vi "Populate Menu Activation.vi"(8 "error in (no error)":errorcluster, 9 "Coords":T1, 10 "MenuRef":refnum<k9>, 11 "Selector in":refnum<class "Selector.lvclass">) -> (0 "error out":errorcluster, 3 "Selector out":refnum<class "Selector.lvclass">)   [LabVIEW 2019, in "Selector.lvclass"]
uses:
  Selector.lvclass
  <vilib>/Utility/miscctls.llb/LVPoint32TypeDef.ctl
  Selector.lvclass/Selector.ctl
  f1f0a02b-b8b6-4cc5-b4ed-f95812147d19.vi
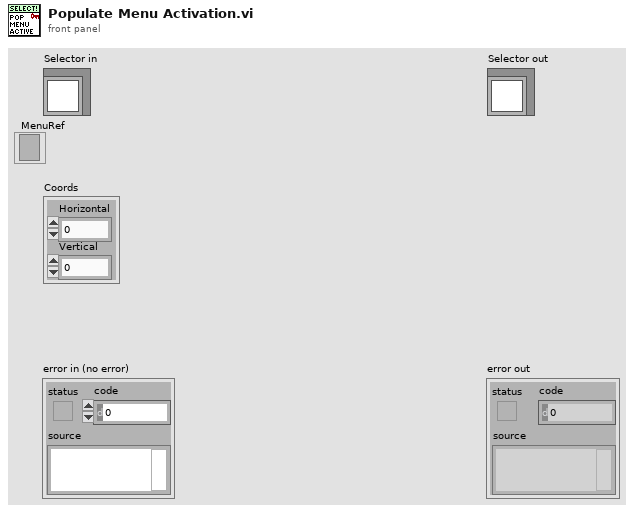
[diagram p1: front panel]
types:
  T1 = typedef "LVPoint32TypeDef.ctl" = cluster{"Horizontal":i32, "Vertical":i32}
  T2 = typedef "Selector.lvclass/Item.ctl" = cluster{"Name":string, "Group":string, "Enabled":bool}
  T3 = typedef "LVRowAndColumnTypeDef.ctl" = cluster{"Row":i32, "Column":i32}
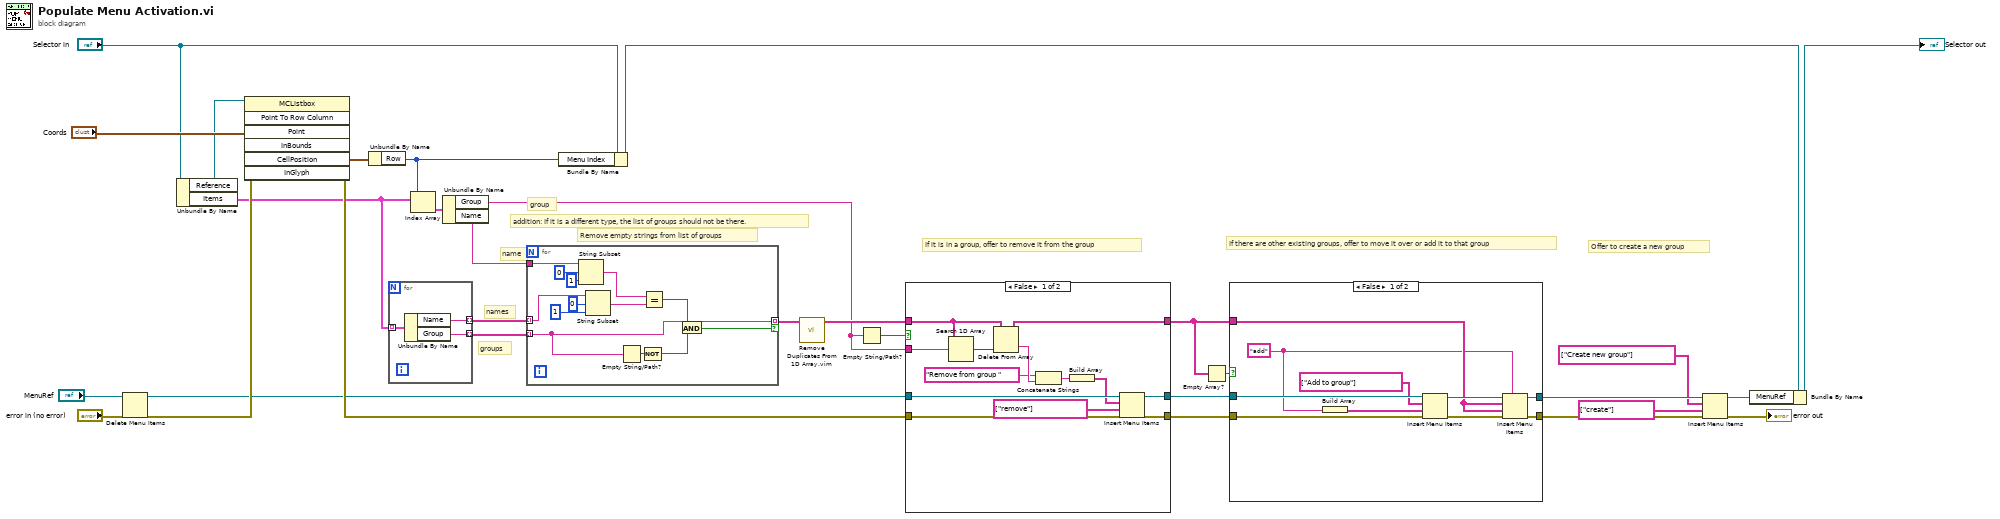
[diagram p0: block diagram]
diagram:
  # "group"
  # "name"
  # "groups"
  # "names"
  # "Remove empty strings from list of groups"
  # "addition: If it is a different type, the list of groups should not be there."
  # "Offer to create a new group"
  # "If there are other existing groups, offer to move it over or add it to that group"
  # "If it is in a group, offer to remove it from the group"
  n1 = Delete Menu Items(6:"error in (no error)", 9:"MenuRef") -> (0:w27:errorcluster, 3:w24:refnum<k9>)  [unwired: 2 in]
  n2 = Unbundle By Name("Selector in") -> ("Reference"=w14:refnum<vi>, "Items"=w3:T2[])
  n3 = invoke class="MCListbox" method="Point To Row Column"(reference=w14, error in=w27, "Point"="Coords") -> (error out=w25:errorcluster, "CellPosition"=w28:T3)  [unwired: 4 in, 5 out]
  n4 = Unbundle By Name(w28) -> ("Row"=w7:i32)
  n5 = for {
    tunnel: w3 -> [w34] mode=indexing
    tunnel: [w33] -> w2 mode=indexing
    tunnel: [w32] -> w1 mode=indexing
    n6 = Unbundle By Name(w34) -> ("Name"=w33:string, "Group"=w32:string)
  }
  n7 = Index Array(array=w3, index=w7) -> (element=w6:T2)
  n8 = Unbundle By Name(w6) -> ("Group"=w4:string, "Name"=w5:string)
  n9 = for {
    tunnel: w5 -> [w47]
    tunnel: [w36] -> w8 mode=indexing if=w35
    tunnel: w2 -> [w38] mode=indexing
    tunnel: w1 -> [w36] mode=indexing
    n10 = String Subset(string=w47, offset (0)=0, length (rest)=1 ("length (rest)")) -> (substring=w41:string)
    n11 = String Subset(string=w38, offset (0)=0, length (rest)=1 ("length (rest)")) -> (substring=w42:string)
    n12 = Empty String/Path?(string/path=w36) -> (empty?=w40:bool)
    n13 = Not(x=w40) -> (.not. x?=w39:bool)
    n14 = Equal?(x=w41, y=w42) -> (x = y?=w37:bool)
    n15 = And(x=w37, y=w39) -> (x .and. y?=w35:bool)
  }
  n16 = Bundle By Name(cluster="Selector in", "Menu Index"=w7) -> (w11:refnum<class "Selector.lvclass">)
  n17 = call "Remove Duplicates From 1D Array.vim"("array"=w8) -> ("array with duplicates removed"=w9:string[])  [unwired: 10 in]
  n18 = Empty String/Path?(string/path=w4) -> (empty?=w26:bool)
  n19 = case shown="False" w26 {
    tunnel: w9 -> [w59 w63]
    tunnel: w4 -> [w60 _]
    tunnel: [w50 w63] -> w20
    tunnel: w25 -> [w53 w61]
    tunnel: [w52 w61] -> w22
    tunnel: w24 -> [w57 w62]
    tunnel: [w51 w62] -> w23
    frame False {
      n20 = Search 1D Array(1D array=w59, element=w60) -> (index of element=w58:i32)  [unwired: 1 in]
      n21 = Delete From Array(array=w59, index=w58) -> (deleted portion=w56:string, array with subset deleted=w50:string[])  [unwired: 1 in]
      n22 = Concatenate Strings("Remove from group " ("string"), w56) -> (w55:string)
      n23 = Build Array(w55) -> (w48:string[])
      n24 = Insert Menu Items(6:w53, 7:string[] ["remove"] ("item tags"), 8:w48, 9:w57) -> (0:w52:errorcluster, 3:w51:refnum<k9>)  [unwired: 2 in, 1 out]
    }
    frame True {
    }
  }
  n25 = Empty Array?(array=w20) -> (empty?=w21:bool)
  n26 = case shown="False" w21 {
    tunnel: w23 -> [w73 w75]
    tunnel: w22 -> [w72 w74]
    tunnel: [w69 w74] -> w17
    tunnel: w20 -> [w68 _]
    tunnel: [w67 w75] -> w19
    frame False {
      w64 = "add" ("menu tag")
      n27 = Build Array(w64) -> (w66:string[])
      n28 = Insert Menu Items(6:w72, 7:w66, 8:string[] ["Add to group"] ("item names"), 9:w73) -> (0:w70:errorcluster, 3:w71:refnum<k9>)  [unwired: 2 in, 1 out]
      n29 = Insert Menu Items(5:w64, 6:w70, 7:w68, 8:w68, 9:w71) -> (0:w69:errorcluster, 3:w67:refnum<k9>)  [unwired: 1 in, 1 out]
    }
    frame True {
    }
  }
  n30 = Insert Menu Items(6:w17, 7:string[] ["create"] ("item tags"), 8:string[] ["Create new group"] ("item names"), 9:w19) -> (0:→"error out":errorcluster, 3:w12:refnum<k9>)  [unwired: 2 in, 1 out]
  n31 = Bundle By Name(cluster=w11, "MenuRef"=w12) -> (→"Selector out":refnum<class "Selector.lvclass">)
